vi "set HO UL_DL Center Channel Number.vi"(8 "error in (no error)":errorcluster caption="에러 입력(에러 없음)", 9 "Direction":T1, 10 "Center Channel Argements":T2, 11 "NR 입력":refnum<class "NR.lvclass">) -> (0 "error out":errorcluster caption="에러 출력", 3 "NR 출력":refnum<class "NR.lvclass">)   [LabVIEW 2023, in "ANRITSU Call Box.lvlib" / "NR.lvclass"]
uses:
  NR.lvclass
  NR.lvclass/NR.ctl
  Type Definition/Uplink Downlink Enum.ctl
  ANRITSU Call Box.lvlib
  Type Definition/NR Center Channel Arguments.ctl
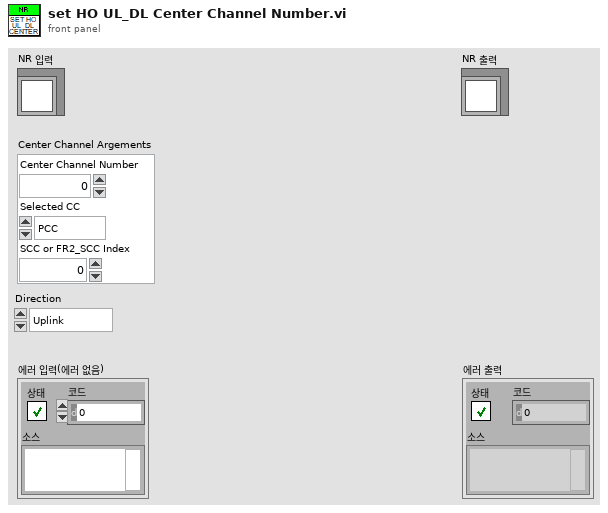
[diagram p1: front panel]
types:
  T1 = typedef "ANRITSU Call Box.lvlib/Uplink Downlink Enum.ctl" = enum16{"Uplink", "Downlink"}
  T2 = typedef "ANRITSU Call Box.lvlib/NR Center Channel Arguments.ctl" = cluster{"Center Channel Number":u32, "Selected CC":enum16{"PCC", "SCC", "FR2_PCC", "FR2_SCC"}, "SCC or FR2_SCC Index":u32}
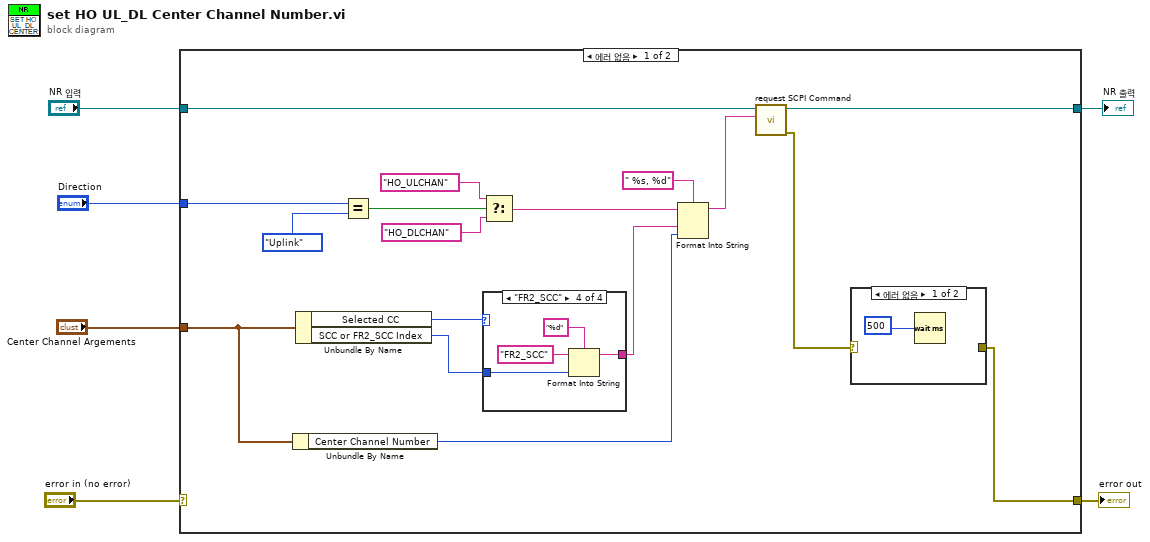
[diagram p0: block diagram]
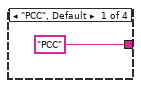
[diagram p3: hidden frame]
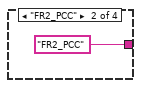
[diagram p4: hidden frame]
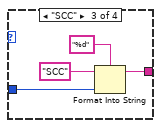
[diagram p5: hidden frame]
diagram:
  n1 = case shown="에러 없음" "error in (no error)" {
    selector: "error in (no error)" -> [_ w37]
    tunnel: [w8 w37] -> w5
    tunnel: [w12 w36] -> w3
    tunnel: "NR 입력" -> [w13 w36]
    tunnel: "Center Channel Argements" -> [w11 _]
    tunnel: "Direction" -> [w9 _]
    frame No Error {
      n2 = Unbundle By Name(w11) -> ("Center Channel Number"=w10:u32)
      n3 = Unbundle By Name(w11) -> ("Selected CC"=w7:enum16{"PCC", "SCC", "FR2_PCC", "FR2_SCC"}, "SCC or FR2_SCC Index"=w19:u32)
      n4 = Equal?(x=w9, y=Uplink_Downlink_Enum."Uplink") -> (x = y?=w20:bool)
      n5 = case shown="\"FR2_SCC\"" w7 {
        tunnel: ["PCC" "FR2_PCC" w29 w33] -> w16
        tunnel: w19 -> [_ _ w28 w32]
        frame "PCC", Default {
        }
        frame "FR2_PCC" {
        }
        frame "SCC" {
          n6 = Format Into String(format string="%d", initial string="SCC", w28) -> (resulting string=w29:string)  [unwired: 1 in, 1 out]
        }
        frame "FR2_SCC" {
          n7 = Format Into String(format string="%d", initial string="FR2_SCC", w32) -> (resulting string=w33:string)  [unwired: 1 in, 1 out]
        }
      }
      n8 = Select(t="HO_ULCHAN", s=w20, f="HO_DLCHAN") -> (s? t:f=w17:string)
      n9 = Format Into String(format string=" %s, %d", initial string=w17, w16, w10) -> (resulting string=w15:string)  [unwired: 1 in, 1 out]
      n10 = call "request SCPI Command.vi"("SCPI Command"=w15, "NR in"=w13) -> ("error out"=w14:errorcluster, "NR out"=w12:refnum<class "NR.lvclass">)  [unwired: 8 in]
      n11 = case shown="에러 없음" w14 {
        selector: w14 -> [_ w25]
        tunnel: [_ w25] -> w8
        frame No Error {
          n12 = Wait (ms)(milliseconds to wait=u32 500) -> ()  [unwired: 1 out]
        }
        frame Error {
        }
      }
    }
    frame Error {
    }
  }
  "error out" <- w5
  "NR 출력" <- w3
